vi "Group Status.vi"(4 "Log Group":T1, 5 "Groups":cluster{"Group":string, "State":string}[](array[cluster])) -> (6 "Group Status":T4, 7 "Group":T1)   [LabVIEW 2020, in "VolatusGUIElements.lvlib" / "GroupLoggingControl.lvclass"]
uses:
  GroupLoggingControl.lvclass
  Log Group.ctl
  Log Group Status.ctl
  Command Info.ctl
  GroupLoggingControl.lvclass/GroupLoggingControl.ctl
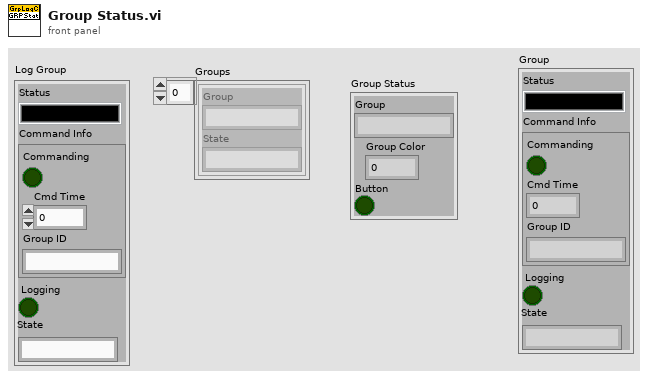
[diagram p1: front panel]
types:
  T1 = typedef "VolatusGUIElements.lvlib/GroupLoggingControl.lvclass/Log Group.ctl" = cluster{"Status":T2, "Command Info":T3, "Logging":bool, "State":string}
  T2 = typedef "VolatusGUIElements.lvlib/GroupLoggingControl.lvclass/Log Group Status.ctl" = cluster{"Group":string, "Group Color":u32, "Button":bool}
  T3 = typedef "VolatusGUIElements.lvlib/GroupLoggingControl.lvclass/Command Info.ctl" = cluster{"Commanding":bool, "Cmd Time":dbl, "Group ID":string}
  T4 = cluster{"Group":string, "Group Color":u32, "Button":bool}
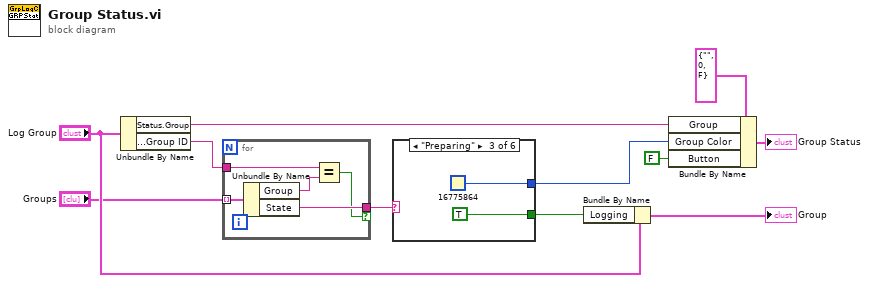
[diagram p0: block diagram]
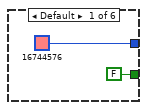
[diagram p2: hidden frame]
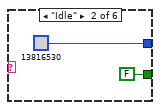
[diagram p3: hidden frame]
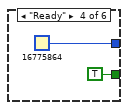
[diagram p4: hidden frame]
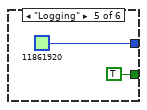
[diagram p5: hidden frame]
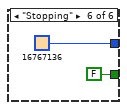
[diagram p6: hidden frame]
diagram:
  n1 = Unbundle By Name("Log Group") -> ("Status.Group"=w3:string, "Command Info.Group ID"=w1:string)
  n2 = for {
    tunnel: "Groups" -> [w16] mode=indexing
    tunnel: w1 -> [w15]
    tunnel: [w13] -> w2 if=w12
    n3 = Unbundle By Name(w16) -> ("Group"=w14:string, "State"=w13:string)
    n4 = Equal?(x=w15, y=w14) -> (x = y?=w12:bool)
  }
  n5 = case shown="\"Preparing\"" w2 {
    tunnel: [u32 16744576 u32 13816530 u32 16775864 u32 16775864 u32 11861920 u32 16767136] -> w9
    tunnel: [FALSE FALSE TRUE TRUE TRUE FALSE] -> w6
    frame Default {
    }
    frame "Idle" {
    }
    frame "Preparing" {
    }
    frame "Ready" {
    }
    frame "Logging" {
    }
    frame "Stopping" {
    }
  }
  n6 = Bundle By Name(cluster="Log Group", "Logging"=w6) -> (→"Group":T1)
  n7 = Bundle By Name(cluster=T4 {"Group"="", "Group Color"=0, "Button"=FALSE} ("Node Status 2"), "Group"=w3, "Group Color"=w9, "Button"=FALSE) -> (→"Group Status":T4)
